vi "RDC-permittivity-error_analysis.vi"(7 "%?":bool, 10 "Analyse":T1, 11 "Correct":T1) -> (0 "AVG imag":dbl, 1 "Perm imag":dbl[](array[numeric]), 2 "AVG Real":dbl, 3 "Perm real":dbl[](array[numeric]))   [LabVIEW 2020, in "RDC-Reflection_Data_Computation.lvlib"]
doc: "Compares the permittivity of the Analyse Common Format cluster with the Correct one. Returns the real and imaginary differences and their averages, as percent when %? is true."
uses:
  RDC-Reflection_Data_Computation.lvlib
  Reflector/RFH-common_data_format.ctl
  3e70a99f-e9bb-40d3-bf36-55773cecfdea.vi
  1fc45e94-24e8-4037-8470-cf1399eea27a.vi
  Reflector/RFH-Reflection_File_Handler.lvlib
panel:
  in  "Analyse 2":T1[](array[typedef])
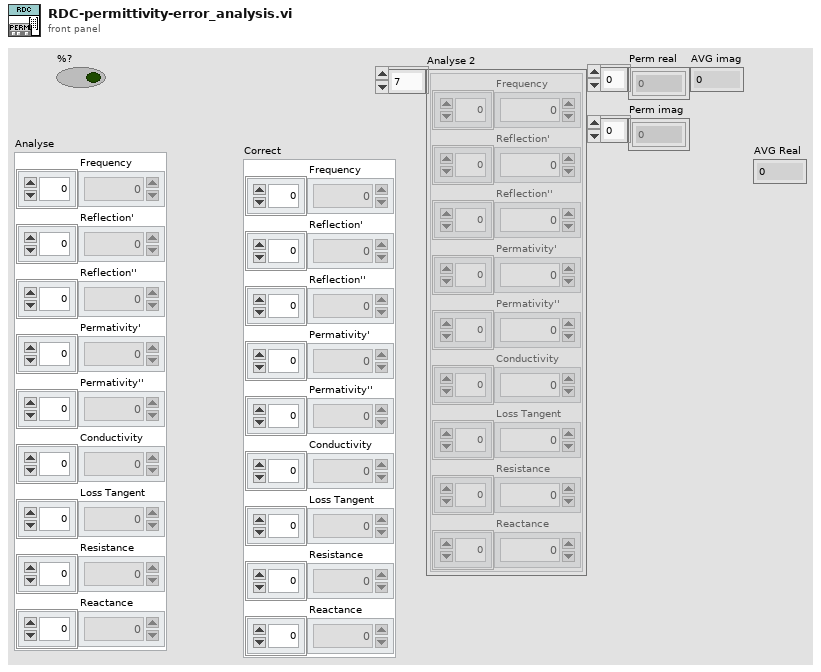
[diagram p1: front panel]
types:
  T1 = typedef "RFH-Reflection_File_Handler.lvlib/RFH-common_data_format.ctl" = cluster{"Frequency":dbl[], "Reflection'":dbl[], "Reflection''":dbl[], "Permativity'":dbl[], "Permativity''":dbl[], "Conductivity":dbl[], "Loss Tangent":dbl[], "Resistance":dbl[], "Reactance":dbl[]}
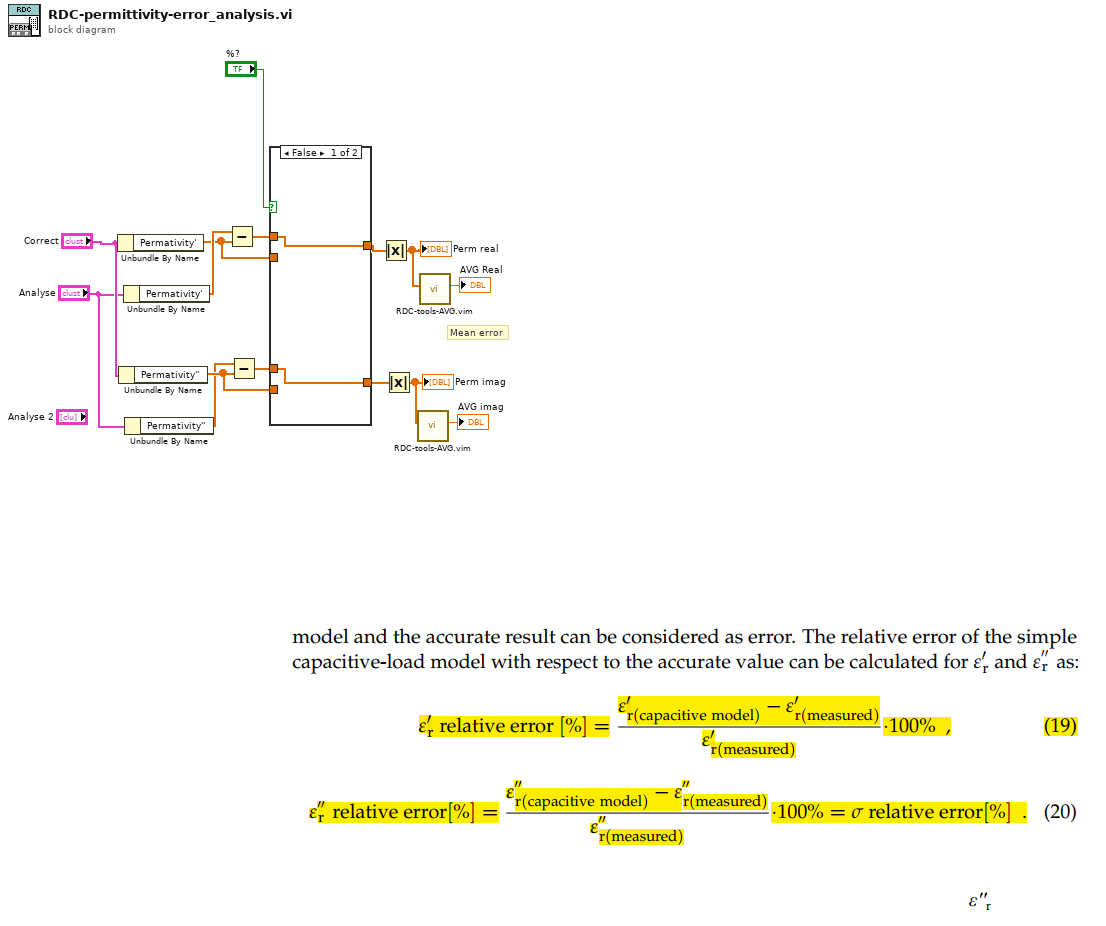
[diagram p0: block diagram]
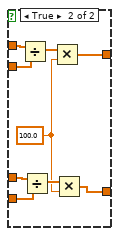
[diagram p2: hidden frame]
diagram:
  # "Mean error"
  n1 = Unbundle By Name("Correct") -> ("Permativity'"=w13:dbl[])
  n2 = Unbundle By Name("Correct") -> ("Permativity''"=w12:dbl[])
  n3 = Unbundle By Name("Analyse") -> ("Permativity'"=w15:dbl[])
  n4 = Unbundle By Name("Analyse") -> ("Permativity''"=w10:dbl[])
  n5 = Subtract(x=w15, y=w13) -> (x-y=w14:dbl[])
  n6 = Subtract(x=w10, y=w12) -> (x-y=w11:dbl[])
  n7 = case shown="False" "%?" {
    tunnel: w14 -> [w17 w26]
    tunnel: w13 -> [_ w25]
    tunnel: w12 -> [_ w22]
    tunnel: w11 -> [w16 w21]
    tunnel: [w17 w19] -> w7
    tunnel: [w16 w18] -> w6
    frame False {
    }
    frame True {
      w20 = 100.0
      n8 = Divide(x=w26, y=w25) -> (x/y=w24:dbl[])
      n9 = Divide(x=w21, y=w22) -> (x/y=w23:dbl[])
      n10 = Multiply(x=w24, y=w20) -> (x*y=w19:dbl[])
      n11 = Multiply(x=w23, y=w20) -> (x*y=w18:dbl[])
    }
  }
  n12 = Absolute Value(x=w7) -> (abs(x)=w5:dbl[])
  "Perm real" <- w5
  n13 = Absolute Value(x=w6) -> (abs(x)=w4:dbl[])
  "Perm imag" <- w4
  n14 = call "RDC-tools-AVG.vim"("Data Array"=w4) -> ("AVG"=→"AVG imag":dbl)  [unwired: 10 in]
  n15 = call "RDC-tools-AVG.vim"("Data Array"=w5) -> ("AVG"=→"AVG Real":dbl)  [unwired: 10 in]
